vi "Execute.vi"(8 "error in (no error)":errorcluster, 11 "Node in":refnum<class "bt_Repeat Until Timeout.lvclass">) -> (0 "error out":errorcluster, 1 "Status":T1, 3 "Node out":refnum<class "bt_Repeat Until Timeout.lvclass">)   [LabVIEW 2021, in "BT.lvlib" / "bt_Repeat Until Timeout.lvclass"]
uses:
  bt_Repeat Until Timeout.lvclass
  abs_Node/Status.ctl
  bt_Repeat Until Timeout.lvclass/bt_Repeat Until Timeout.ctl
  Repeater/bt_Repeater.lvclass
  abs_Node/bt_Node.lvclass
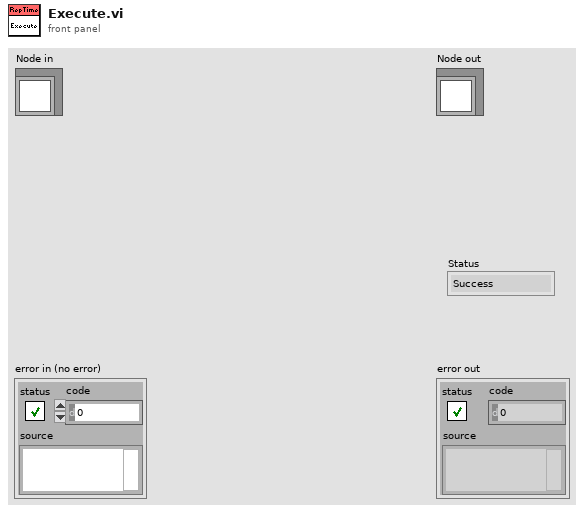
[diagram p1: front panel]
types:
  T1 = typedef "BT.lvlib/bt_Node.lvclass/Status.ctl" = enum16{"Success", "Failure", "Running"}
  T2 = typedef "BT.lvlib/bt_Repeat Until Timeout.lvclass/On Timeout Status - Type.ctl" = enum16{"Success", "Failure"}
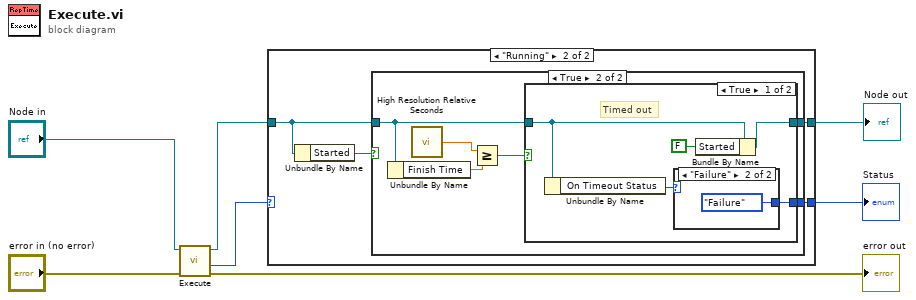
[diagram p0: block diagram]
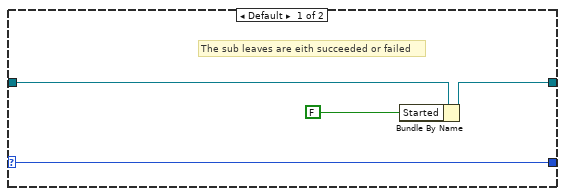
[diagram p2: hidden frame]
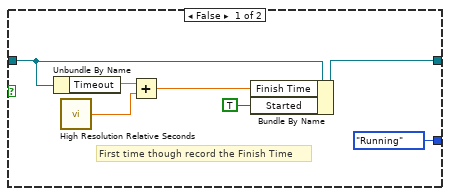
[diagram p3: hidden frame]
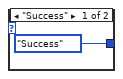
[diagram p4: hidden frame]
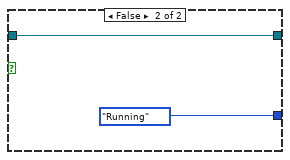
[diagram p5: hidden frame]
diagram:
  n1 = call-parent "Execute.vi"("error in (no error)"="error in (no error)", "Node in"="Node in") -> ("error out"=→"error out":errorcluster, "Status"=w1:T1, "Node out"=w2:refnum<class "bt_Repeat Until Timeout.lvclass">)  [unwired: 7 in]
  n2 = case shown="\"Running\"" w1 {
    selector: w1 -> [w11 _]
    tunnel: w2 -> [w10 w13]
    tunnel: [w11 w14] -> w4
    tunnel: [w9 w15] -> w3
    frame Default {
      # "The sub leaves are eith succeeded or failed"
      n3 = Bundle By Name(cluster=w10, "Started"=FALSE) -> (w9:refnum<class "bt_Repeat Until Timeout.lvclass">)
    }
    frame "Running" {
      n4 = Unbundle By Name(w13) -> ("Started"=w12:bool)
      n5 = case shown="True" w12 {
        tunnel: w13 -> [w20 w28]
        tunnel: [w21 w27] -> w15
        tunnel: [Status."Running" ("Status") w26] -> w14
        frame False {
          # "First time though record the Finish Time"
          n6 = Unbundle By Name(w20) -> ("Timeout"=w19:dbl)
          n7 = call <vilib>:"High Resolution Relative Seconds.vi"() -> ("relative seconds"=w16:dbl)
          n8 = Add(x=w19, y=w16) -> (x+y=w18:dbl)
          n9 = Bundle By Name(cluster=w20, "Finish Time"=w18, "Started"=TRUE) -> (w21:refnum<class "bt_Repeat Until Timeout.lvclass">)
        }
        frame True {
          n10 = Unbundle By Name(w28) -> ("Finish Time"=w25:dbl)
          n11 = call <vilib>:"High Resolution Relative Seconds.vi"() -> ("relative seconds"=w24:dbl)
          n12 = Greater Or Equal?(x=w24, y=w25) -> (x >= y?=w23:bool)
          n13 = case shown="True" w23 {
            tunnel: w28 -> [w31 w37]
            tunnel: [w30 w37] -> w27
            tunnel: [w33 Status."Running" ("Status")] -> w26
            frame True {
              # "Timed out"
              n14 = Unbundle By Name(w31) -> ("On Timeout Status"=w32:T2)
              n15 = case shown="\"Failure\"" w32 {
                tunnel: [Status."Success" ("Status") Status."Failure" ("Status")] -> w33
                frame "Success" {
                }
                frame "Failure" {
                }
              }
              n16 = Bundle By Name(cluster=w31, "Started"=FALSE) -> (w30:refnum<class "bt_Repeat Until Timeout.lvclass">)
            }
            frame False {
            }
          }
        }
      }
    }
  }
  "Node out" <- w3
  "Status" <- w4
